vi "Enable Drive.vi"(8 "error in (no error)":errorcluster, 10 "Enable Drive":bool, 11 "WEG_SCA06_Modbus in":refnum<class "WEG_SCA06_Modbus.lvclass">) -> (0 "error out":errorcluster, 3 "WEG_SCA06_Modbus out":refnum<class "WEG_SCA06_Modbus.lvclass">)   [LabVIEW 2021, in "WEG_SCA06_Modbus.lvclass"]
uses:
  WEG_SCA06_Modbus.lvclass
  WEG_SCA06_Modbus.lvclass/WEG_SCA06_Modbus.ctl
  Modbus_Master/Modbus_Master.lvclass
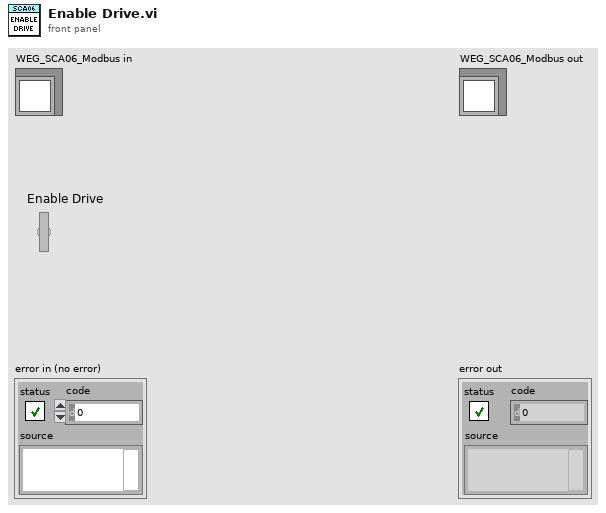
[diagram p1: front panel]
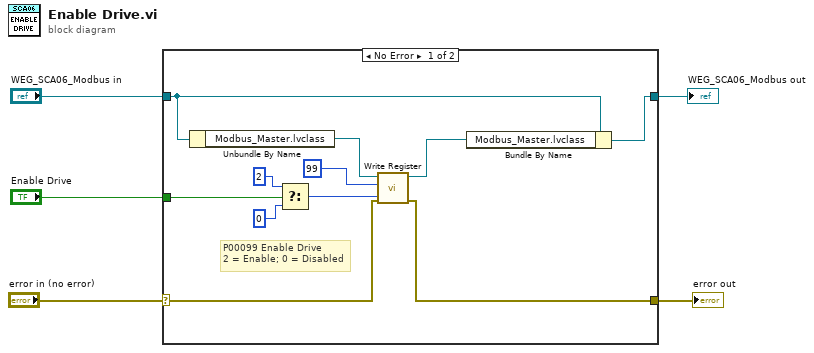
[diagram p0: block diagram]
diagram:
  n1 = case shown="No Error" "error in (no error)" {
    selector: "error in (no error)" -> [w7 w18]
    tunnel: "Enable Drive" -> [w11 _]
    tunnel: "WEG_SCA06_Modbus in" -> [w15 w17]
    tunnel: [w16 w17] -> w2
    tunnel: [w6 w18] -> w1
    frame No Error {
      # "P00099 Enable Drive\n2 = Enable; 0 = Disabled"
      n2 = Unbundle By Name(w15) -> ("Modbus_Master.lvclass"=w14:refnum<class "Modbus_Master.lvclass">)
      n3 = Select(t=u16 2 ("Register Address"), s=w11, f=u16 0 ("Register Address")) -> (s? t:f=w8:u16)
      n4 = call "Write Register.vi"("error in (no error)"=w7, "Value"=w8, "Register Address"=u16 99, "Modbus_Master in"=w14) -> ("error out"=w6:errorcluster, "Modbus_Master out"=w13:refnum<class "Modbus_Master.lvclass">)  [unwired: 6 in]
      n5 = Bundle By Name(cluster=w15, "Modbus_Master.lvclass"=w13) -> (w16:refnum<class "WEG_SCA06_Modbus.lvclass">)
    }
    frame Error {
    }
  }
  "error out" <- w1
  "WEG_SCA06_Modbus out" <- w2
